vi "sftpdir.vi"() -> ()   [LabVIEW 2017]
doc: "This example illustrates SFTP directory listing."
uses:
  libssh2/libssh2_session_handshake_tcp.vi
  libssh2/libssh2_init_default.vi
  libssh2/libssh2_session_init_ex.vi
  <vilib>/Utility/tcp.llb/TCP Get Raw Net Object.vi
  libssh2/libssh2_session_handshake_socket.vi
  libssh2/libssh2_userauth_password_ex.vi
  libssh2/libssh2_sftp_open_ex.vi
  libssh2/libssh2.lvlib
panel:
  in  "directory":string="/"
  out "individual files":string[](array[string])
  out "directory listing":string
  out "error out":errorcluster
  in  "password":string
  in  "username":string
  in  "hostname":string
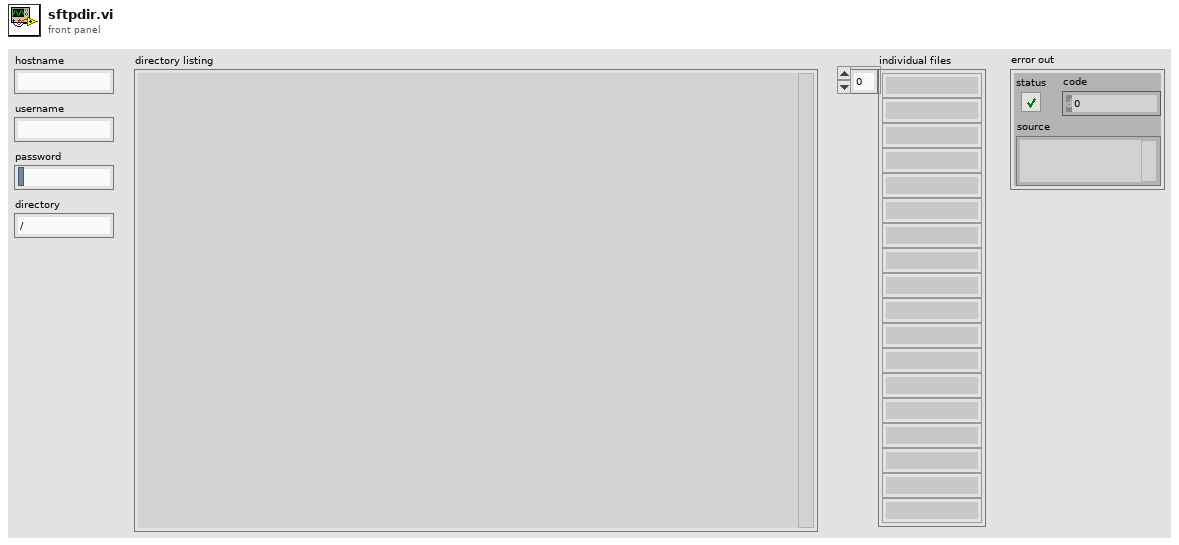
[diagram p1: front panel]
types:
  T1 = typedef "libssh2.lvlib/Session Refnum.ctl" = refnum<k1>
  T2 = typedef "libssh2.lvlib/SFTP Refnum.ctl" = refnum<k1>
  T3 = typedef "libssh2.lvlib/SFTP Handle Refnum.ctl" = refnum<k1>
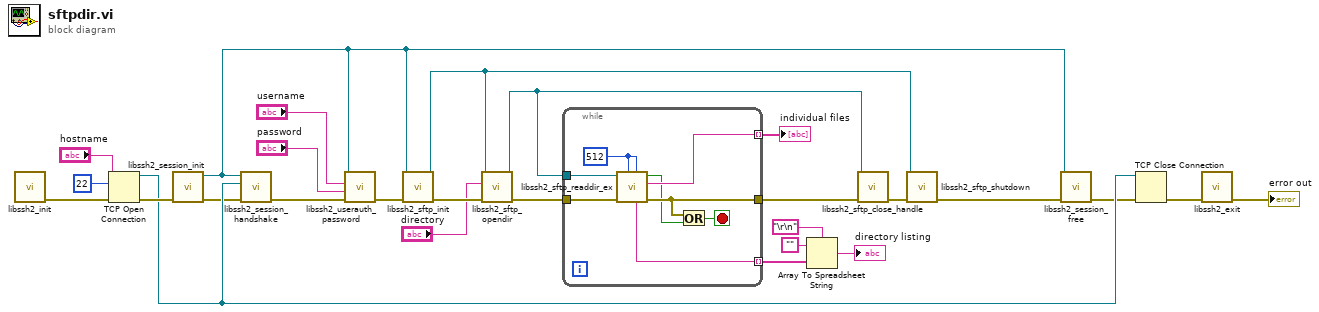
[diagram p0: block diagram]
diagram:
  n1 = call-poly "libssh2_init.vi"() -> ("error out"=w27:errorcluster)  [unwired: 11 in]
  n2 = TCP Open Connection(address="hostname", remote port or service name=u16 22, error in (no error)=w27) -> (connection ID=w25:refnum<k5>, error out=w26:errorcluster)  [unwired: 2 in]
  n3 = call "libssh2_session_init.vi"("error in (no error)"=w26) -> ("error out"=w24:errorcluster, "session"=w2:T1)  [unwired: 9 in]
  n4 = call-poly "libssh2_session_handshake.vi"("error in (no error)"=w24, "tcp connection"=w25, "session"=w2) -> ("error out"=w1:errorcluster)  [unwired: 8 in]
  n5 = call "libssh2_userauth_password.vi"("error in (no error)"=w1, "password"="password", "username"="username", "session"=w2) -> ("error out"=w21:errorcluster)  [unwired: 7 in]
  n6 = call "libssh2_sftp_init.vi"("error in (no error)"=w21, "session"=w2) -> ("error out"=w14:errorcluster, "sftp"=w12:T2)  [unwired: 8 in]
  n7 = call "libssh2_sftp_opendir.vi"("error in (no error)"=w14, "path"="directory", "sftp"=w12) -> ("error out"=w13:errorcluster, "sftp handle"=w8:T3)  [unwired: 7 in]
  n8 = while {
    tunnel: w13 -> [w35]
    tunnel: [w31] -> w9
    tunnel: w8 -> [w34]
    tunnel: [w28] -> w6 mode=indexing
    tunnel: [w32] -> w3 mode=indexing
    stop <- w29 stop-if-true
    w33 = 512 ("buffer maxlen")
    n9 = call "libssh2_sftp_readdir_ex.vi"("longentry maxlen (0)"=w33, "buffer maxlen"=w33, "error in (no error)"=w35, "sftp handle"=w34) -> ("error out"=w31:errorcluster, "buffer"=w32:string, "no more files"=w30:bool, "longentry"=w28:string)  [unwired: 3 in, 1 out]
    n10 = Or(x=w31, y=w30) -> (x .or. y?=w29:bool)
  }
  "individual files" <- w3
  n11 = Array To Spreadsheet String(delimiter (Tab)="\r\n", array=w6, 3:"" ("format string")) -> (spreadsheet string=→"directory listing":string)
  n12 = call "libssh2_sftp_close_handle.vi"("error in (no error)"=w9, "sftp handle"=w8) -> ("error out"=w10:errorcluster)  [unwired: 9 in]
  n13 = call "libssh2_sftp_shutdown.vi"("error in (no error)"=w10, "sftp"=w12) -> ("error out"=w15:errorcluster)  [unwired: 9 in]
  n14 = call "libssh2_session_free.vi"("error in (no error)"=w15, "session"=w2) -> ("error out"=w17:errorcluster)  [unwired: 9 in]
  n15 = TCP Close Connection(connection ID=w25, error in (no error)=w17) -> (error out=w16:errorcluster)  [unwired: 1 in, 1 out]
  n16 = call "libssh2_exit.vi"("error in (no error)"=w16) -> ("error out"=→"error out":errorcluster)  [unwired: 10 in]
